vi "Main.vi"() -> ()   [LabVIEW 2026]
uses:
  <vilib>/Instr/_visa.llb/VISA Configure Serial Port (Instr).vi
panel:
  out "SR MODO":enum16{"AUTOMATICO", "MANUAL"}(ring)=enum."MANUAL"
  out "Boton Reset":string
  out "Errores CRC":dbl
  out "Tramas OK":dbl
  out "Estado":string
  out "SALIDA PWM":dbl(graph)
  in  "MODO":bool=TRUE
  in  "RESET":bool
  out "Maquina":T1(ring)
  in  "EMERGENCIA":bool
  in  "PWM":dbl min=0.0 max=100.0
  out "SP Vs ALTURA":cluster{dbl, dbl}(graph)
  out "PING PONG":dbl(slide) scale=0.0..50.0
  out "PID":T2(ring)
  out "error out":errorcluster
  out "Enum":enum16{"DESCONECTADO", "CONECTADO"}(ring)
  out "ESTADO  SYS":enum16{"DETENIDO", "EJECUTANDO", "ERROR"}(ring)
  in  "PARADA":bool
  in  "INICIO":bool
  out "PID":string
  in  "SP":dbl=25.0 min=0.0 max=100.0
  in  "KD":dbl=0.07 min=0.0 max=65535.0
  in  "KI":dbl=0.14 min=0.0 max=65535.0
  in  "KP":dbl=3.9 min=0.0 max=65535.0
  in  "PID":bool
  out "PWM":dbl format="%.2g"
  out "ERROR":dbl format="%.2g"
  out "ALTURA":dbl format="%.2g"
  out "SP":dbl format="%.2f"
  out "array":string[][](array[string])
  out "Procesar":string
  in  "Stop Simulation":bool
  in  "Numeric":u32=115200
  in  "VISA resource name":refnum<visa-resource-name>="COM12"
  out "Iteracion":i32
  # "Sistema Levitador Neumático"
  # "Planta"
  # "Grafico en Tiempo Real"
  # "COMUNICACIÓN"
  # "ESTADO DEL SISTEMA"
  # "Estado :"
  # "Puerto :"
  # "Comunicación :"
  # "Baud :"
  # "Estado PID :"
  # "CONFIGURACIÓN PID"
  # "VARIABLES EN TIEMPO REAL"
  # "KP :"
  # "KI :"
  # "KD :"
  # "AUTO"
  # "MANUAL"
  # "SP :"
  # "PWM :"
  # "Mensaje a Procesar :"
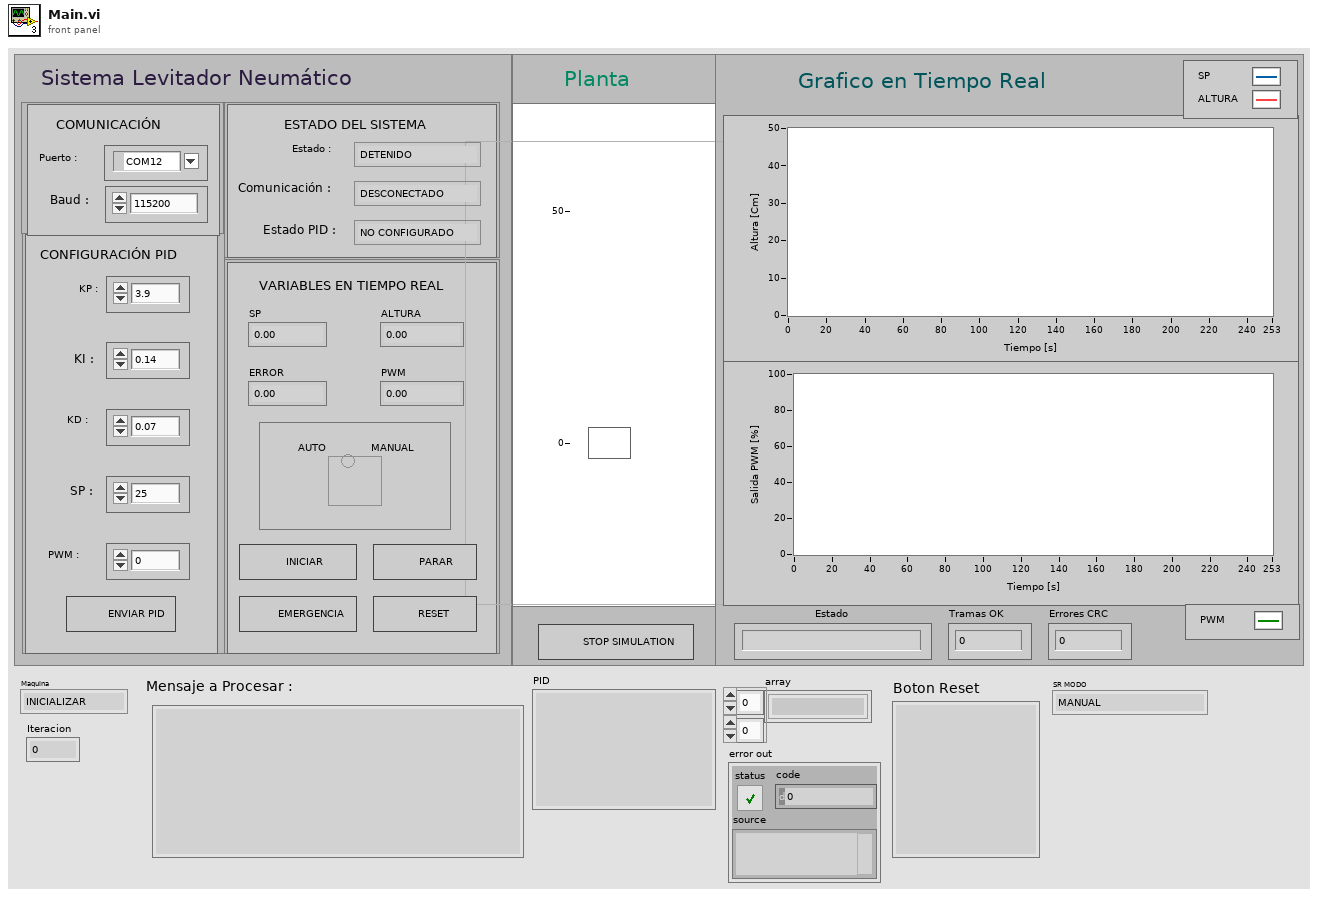
[diagram p1: front panel]
types:
  T1 = enum16{"INICIALIZAR", "ESPERA", "ENVIAR_MODO", "ENVIAR_SP", "ENVIAR_PID", "RECIBIR", "PROCESAR", "ENVIAR_RESET", "ENVIAR_RUN", "ENVIAR_STOP", "ENVIAR_EMERGENCIA_ON", "ENVIAR_EMERGENCIA_OFF", "ERROR", "CERRAR"}
  T2 = enum16{"NO CONFIGURADO", "CONFIGURADO", "AUTOMATICO"}
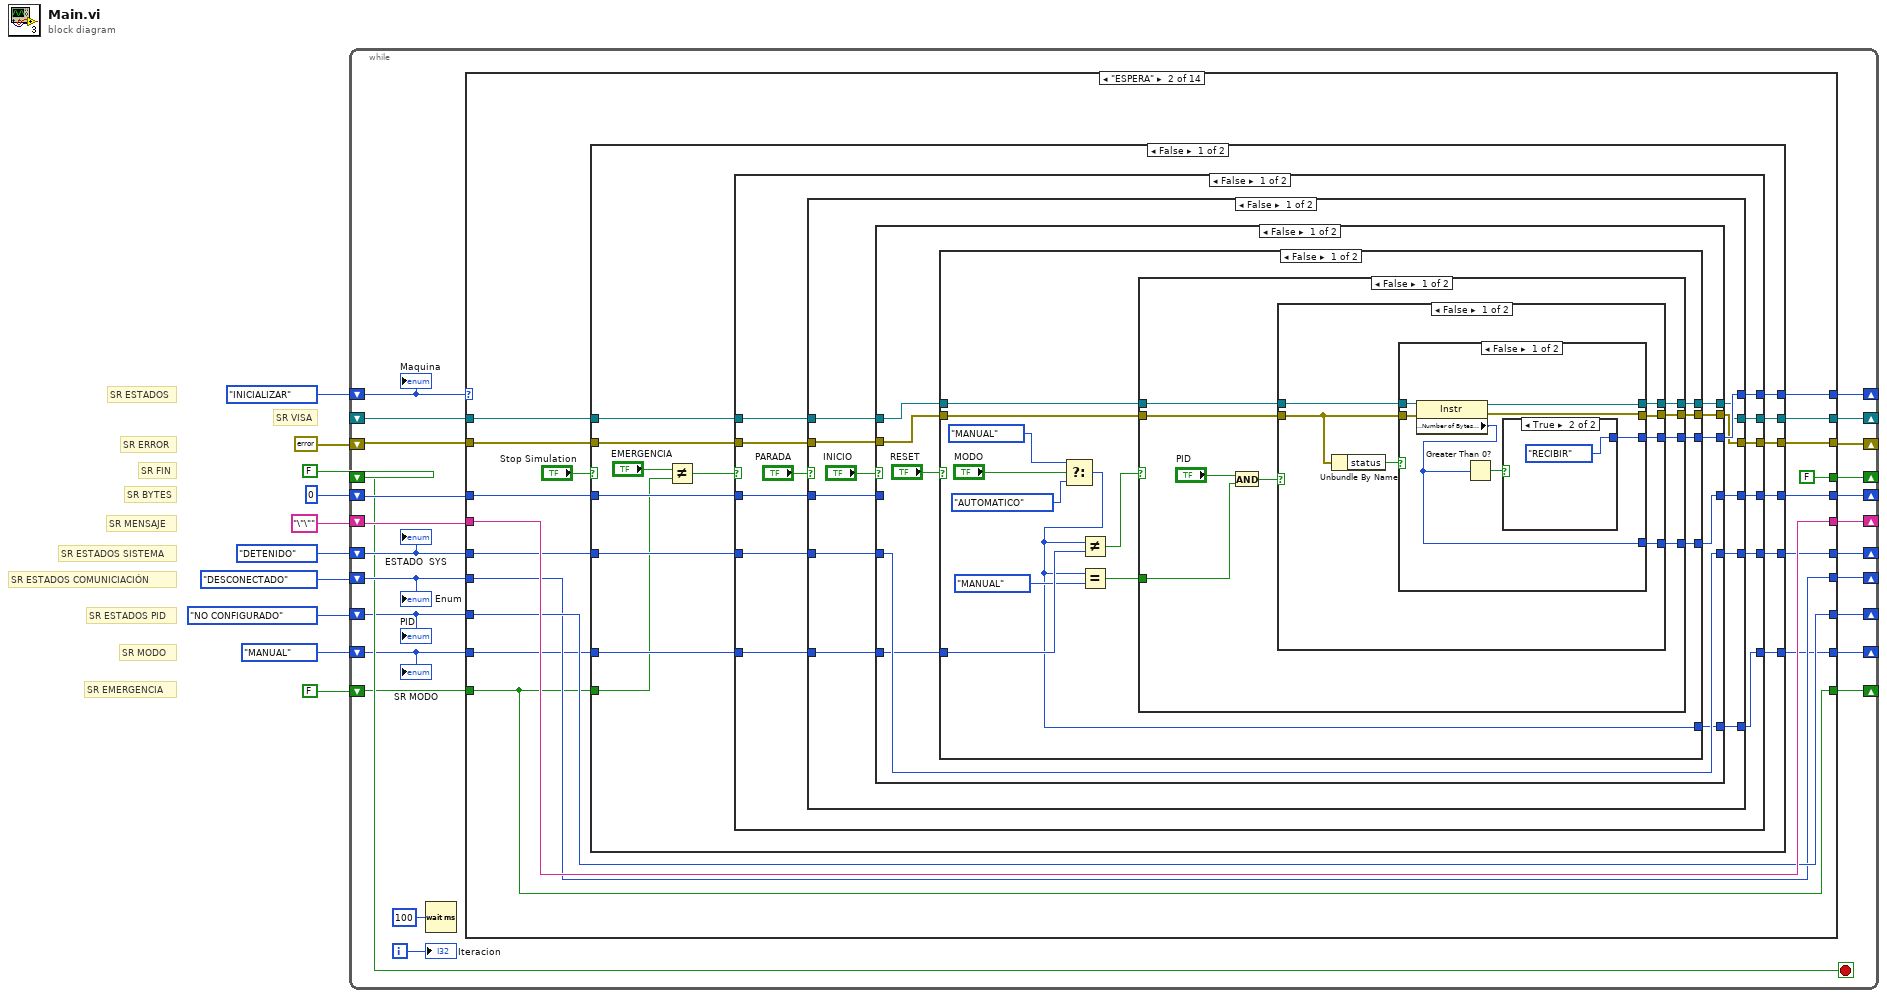
[diagram p0: block diagram]
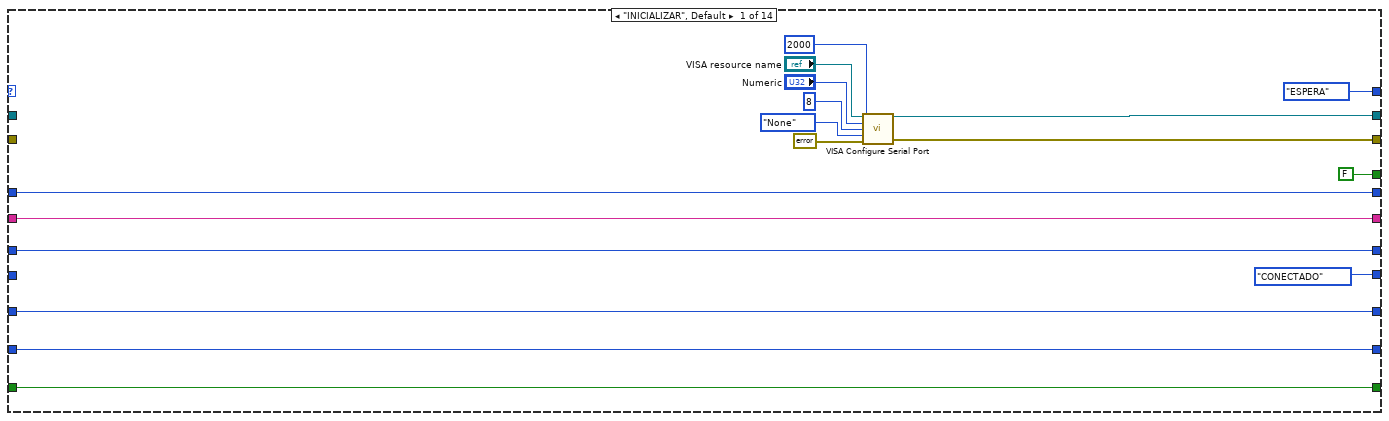
[diagram p2: hidden frame]
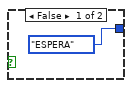
[diagram p3: hidden frame]
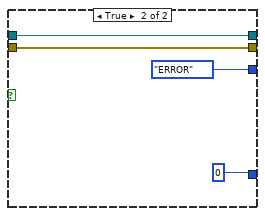
[diagram p4: hidden frame]
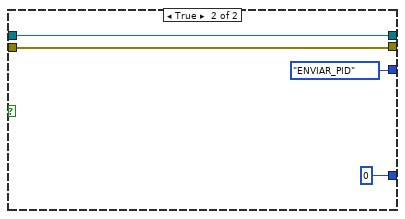
[diagram p5: hidden frame]
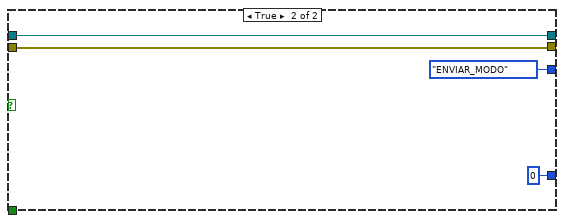
[diagram p6: hidden frame]
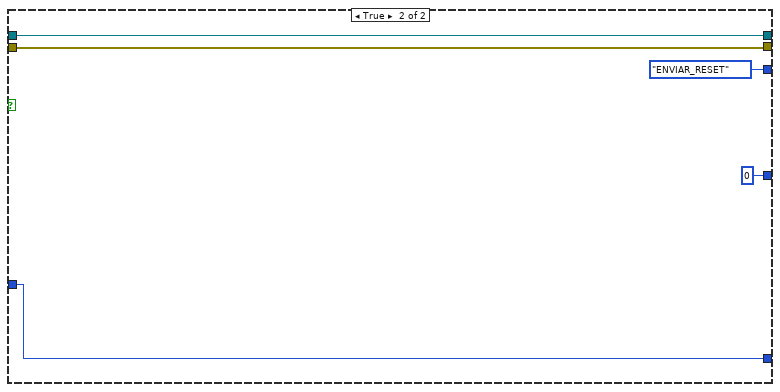
[diagram p7: hidden frame]
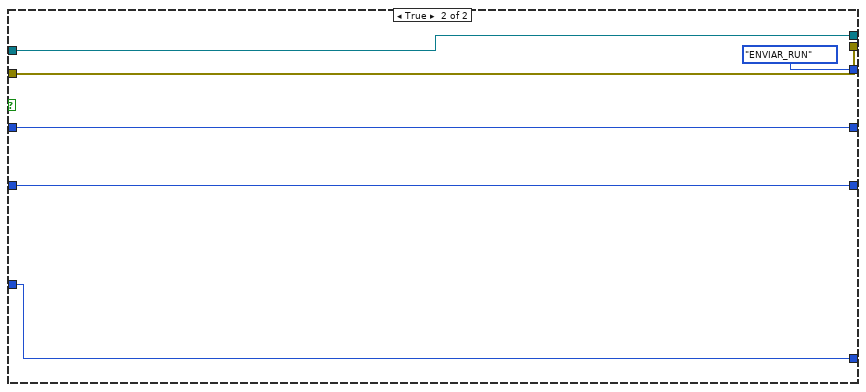
[diagram p8: hidden frame]
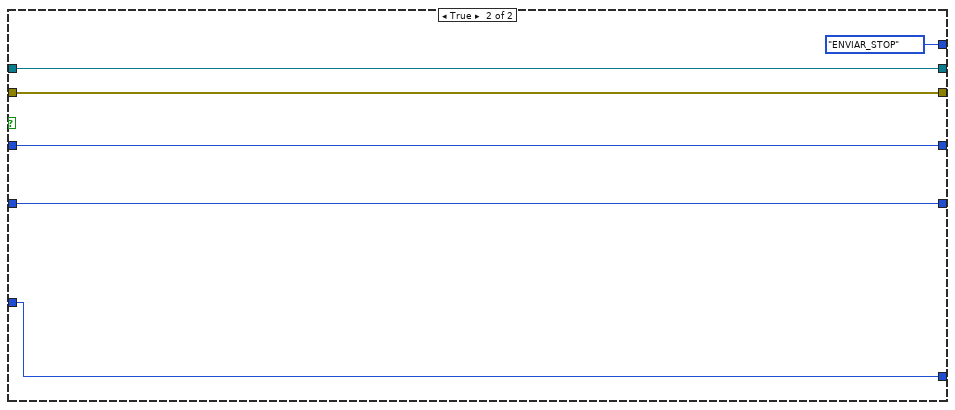
[diagram p9: hidden frame]
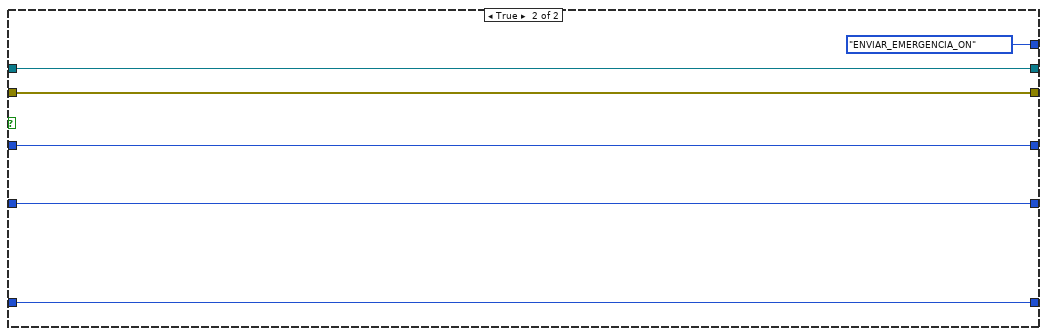
[diagram p10: hidden frame]
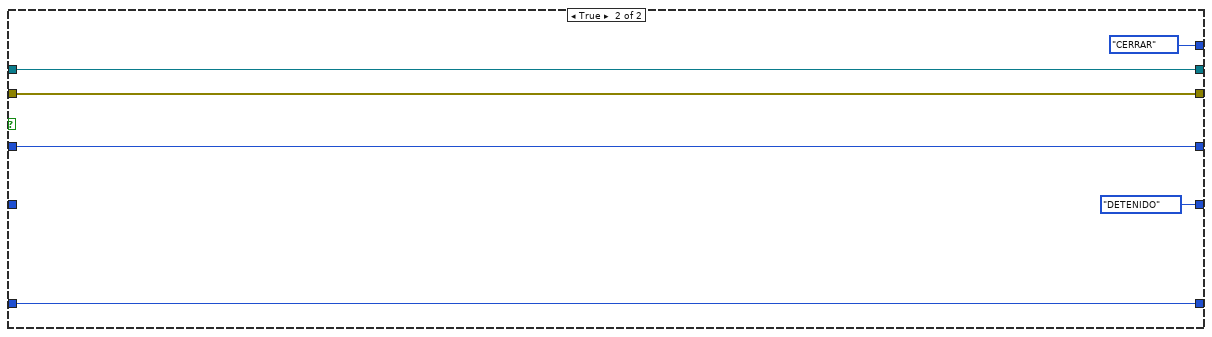
[diagram p11: hidden frame]
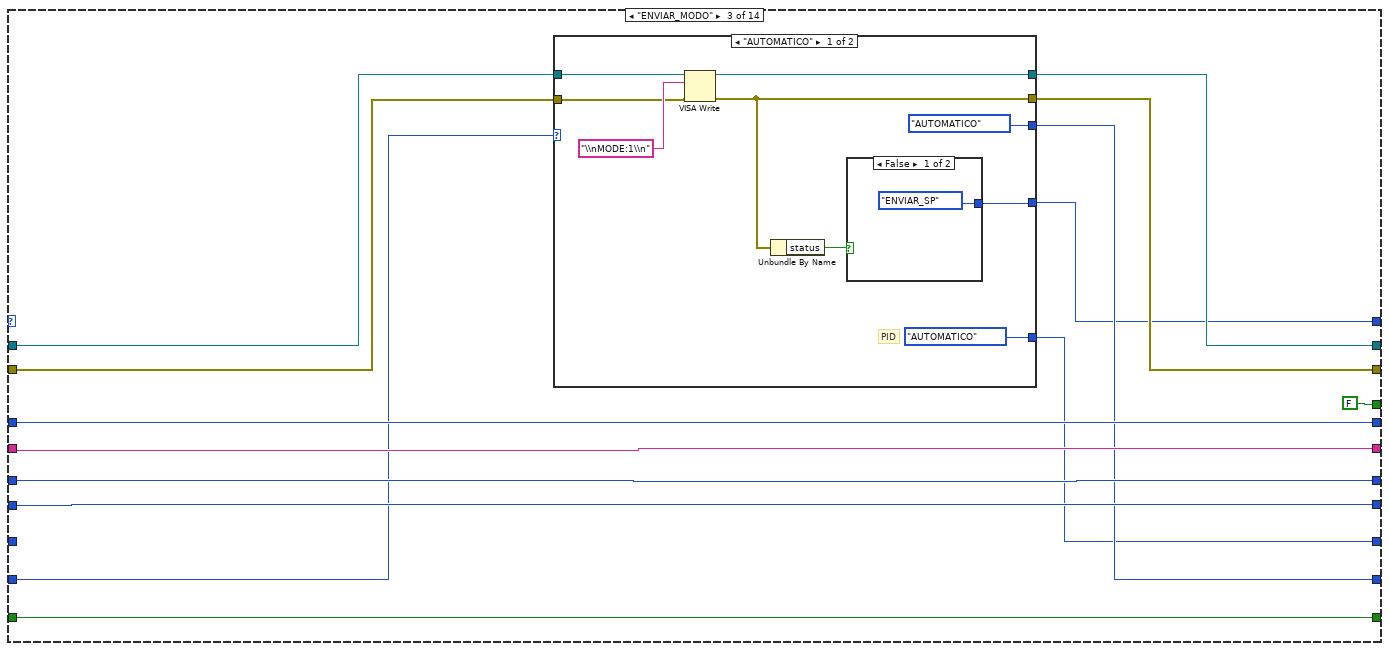
[diagram p12: hidden frame]
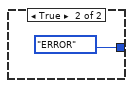
[diagram p13: hidden frame]
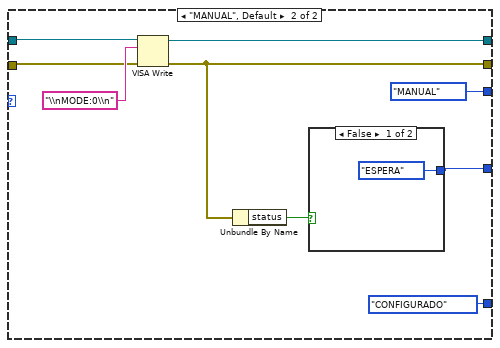
[diagram p14: hidden frame]
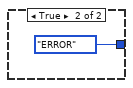
[diagram p15: hidden frame]
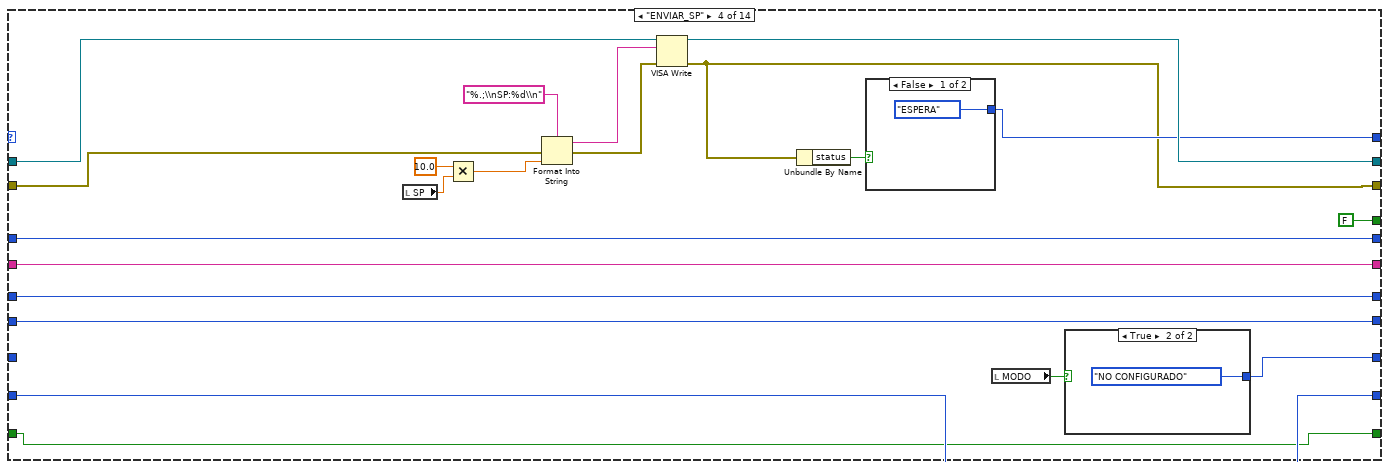
[diagram p16: hidden frame]
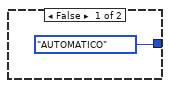
[diagram p17: hidden frame]
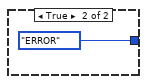
[diagram p18: hidden frame]
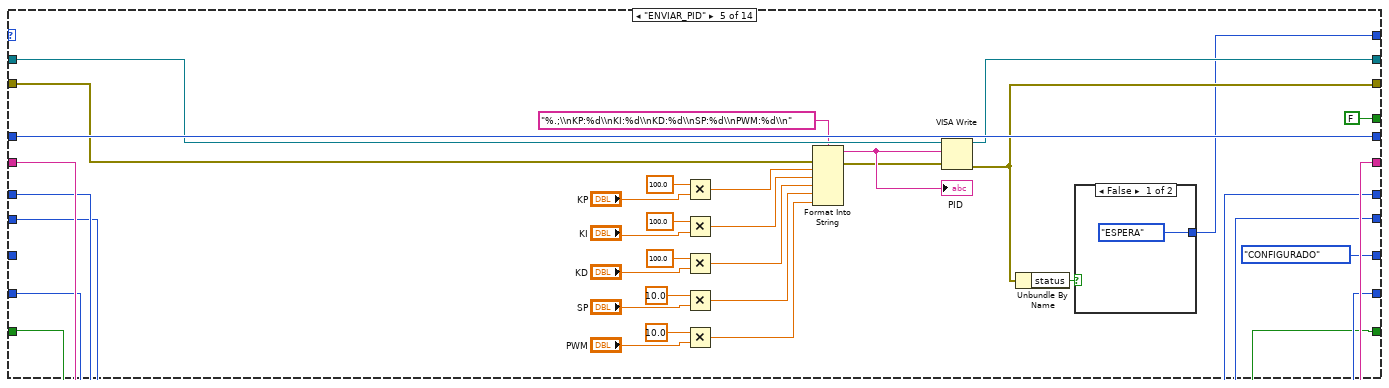
[diagram p19: hidden frame]
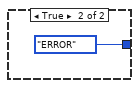
[diagram p20: hidden frame]
diagram:
  # "SR EMERGENCIA"
  # "SR MODO"
  # "SR ESTADOS PID"
  # "SR ESTADOS COMUNICIACIÓN"
  # "SR ESTADOS SISTEMA"
  # "SR MENSAJE"
  # "SR BYTES"
  # "SR FIN"
  # "SR ERROR"
  # "SR ESTADOS"
  # "SR VISA"
  n1 = while {
    shift-right: [w32] -> _
    shift-left: _ -> [w30]
    shift-right: [w31] -> _
    shift-left: errorcluster {"status"=FALSE, "code"=0, "source"=""} ("error out") -> [w29]
    shift-right: [w28] -> _
    shift-left: FALSE -> [w19]
    shift-right: [w27] -> _
    shift-left: u32 0 ("Bytes at Port") -> [w26]
    shift-right: [w25] -> _
    shift-left: "\"\"" -> [w24]
    shift-right: [w20] -> _
    shift-left: enum16{"DETENIDO", "EJECUTANDO", "ERROR"}."DETENIDO" -> [w22]
    shift-right: [w21] -> _
    shift-left: enum16{"DESCONECTADO", "CONECTADO"}."DESCONECTADO" -> [w23]
    shift-right: [w17] -> _
    shift-left: T2."NO CONFIGURADO" -> [w18]
    shift-right: [w15] -> _
    shift-left: T1."INICIALIZAR" -> [w16]
    shift-right: [w13] -> _
    shift-left: enum16{"AUTOMATICO", "MANUAL"}."MANUAL" -> [w14]
    shift-right: [w11] -> _
    shift-left: FALSE -> [w12]
    i -> [w34]
    stop <- w19 stop-if-true
    n2 = Wait (ms)(milliseconds to wait=u32 100) -> ()  [unwired: 1 out]
    n3 = case shown="\"ESPERA\"" w16 {
      tunnel: [T1."ESPERA" w53 w199 w238 w278 w297 T1."ESPERA" w395 w415 w430 w449 w466 T1."CERRAR" T1."CERRAR"] -> w15
      tunnel: [w45 w66 w203 w239 w283 w302 w334 w397 w417 w431 w446 w468 w485 w490] -> w32
      tunnel: [w44 w65 w202 w237 w280 w299 w325 w392 w416 w432 w445 w467 w481 w491] -> w31
      tunnel: w30 -> [_ w67 w205 w241 w284 w304 w334 w399 w419 w436 w451 w470 w485 w490]
      tunnel: w29 -> [_ w61 w204 w240 w286 w303 w326 w398 w418 w435 w450 w469 w481 w492]
      tunnel: [FALSE FALSE FALSE FALSE FALSE FALSE FALSE FALSE FALSE FALSE FALSE FALSE FALSE TRUE] -> w28
      tunnel: [w42 w64 w208 w250 w288 w301 w321 w388 w412 w433 w447 w463 w483 w496] -> w27
      tunnel: w26 -> [w42 w63 w208 w250 w288 w301 w321 w388 w412 w433 w447 w463 w483 w496]
      tunnel: [w41 w62 w209 w251 w287 w300 w319 w394 w413 w434 w444 w462 w482 w495] -> w25
      tunnel: w24 -> [w41 w62 w209 w251 w287 _ w319 w394 w413 w434 w444 w462 w482 w495]
      tunnel: w22 -> [w40 w59 w207 w253 w277 w296 w312 w393 _ _ _ w459 w480 _]
      tunnel: w23 -> [_ w56 w206 w249 w261 w294 w310 w391 w409 w426 w443 w460 w477 _]
      tunnel: [enum16{"DESCONECTADO", "CONECTADO"}."CONECTADO" w56 w206 w249 w261 w294 w310 w391 w409 w426 w443 w460 w477 enum16{"DESCONECTADO", "CONECTADO"}."DESCONECTADO"] -> w21
      tunnel: [w40 w60 w207 w253 w277 w296 w312 w393 enum16{"DETENIDO", "EJECUTANDO", "ERROR"}."EJECUTANDO" enum16{"DETENIDO", "EJECUTANDO", "ERROR"}."DETENIDO" enum16{"DETENIDO", "EJECUTANDO", "ERROR"}."DETENIDO" w459 w480 enum16{"DETENIDO", "EJECUTANDO", "ERROR"}."DETENIDO"] -> w20
      tunnel: w18 -> [w39 w57 _ _ _ w295 w311 _ w410 w427 w448 w464 w479 w489]
      tunnel: [w39 w57 w198 w236 T2."CONFIGURADO" w295 w311 T2."NO CONFIGURADO" w410 w427 w448 w464 w479 w489] -> w17
      tunnel: w14 -> [w36 w55 w200 w234 w259 w293 w309 w389 w408 w425 w442 w461 w476 w487]
      tunnel: [w36 w54 w201 w234 w259 w293 w309 w389 w408 w425 w442 w461 w476 w487] -> w13
      tunnel: w12 -> [w35 w52 w197 w233 w258 w292 w308 w387 w407 w424 _ _ w475 w486]
      tunnel: [w35 w52 w197 w233 w258 w292 w308 w387 w407 w424 TRUE FALSE w475 w486] -> w11
      frame "INICIALIZAR", Default {
        n4 = call-poly "VISA Configure Serial Port"("VISA resource name"="VISA resource name", "timeout (10sec)"=u32 2000, "baud rate (9600)"="Numeric", "data bits (8)"=u16 8, "parity (0:none)"=enum16{"None", "Odd", "Even", "Mark", "Space"}."None", "error in (no error)"=errorcluster {"status"=FALSE, "code"=0, "source"=""}) -> ("VISA resource name out"=w45:refnum<visa-resource-name>, "error out"=w44:errorcluster)  [unwired: 8 in]
      }
      frame "ESPERA" {
        n5 = case shown="False" "Stop Simulation" {
          tunnel: [w82 T1."CERRAR"] -> w53
          tunnel: w67 -> [w81 w194]
          tunnel: [w80 w194] -> w66
          tunnel: [w79 w193] -> w65
          tunnel: [w78 w196] -> w64
          tunnel: w63 -> [w77 w196]
          tunnel: w61 -> [w76 w193]
          tunnel: [w75 enum16{"DETENIDO", "EJECUTANDO", "ERROR"}."DETENIDO"] -> w60
          tunnel: w59 -> [w74 _]
          tunnel: w55 -> [w73 w191]
          tunnel: [w72 w191] -> w54
          tunnel: w52 -> [w69 _]
          frame False {
            n6 = Not Equal?(x="EMERGENCIA", y=w69) -> (x != y?=w70:bool)
            n7 = case shown="False" w70 {
              tunnel: [w94 T1."ENVIAR_EMERGENCIA_ON"] -> w82
              tunnel: w81 -> [w86 w188]
              tunnel: [w93 w188] -> w80
              tunnel: [w92 w187] -> w79
              tunnel: [w91 w190] -> w78
              tunnel: w77 -> [w90 w190]
              tunnel: w76 -> [w85 w187]
              tunnel: [w88 w189] -> w75
              tunnel: w74 -> [w87 w189]
              tunnel: w73 -> [w84 w185]
              tunnel: [w83 w185] -> w72
              frame False {
                n8 = case shown="False" "PARADA" {
                  tunnel: [w106 T1."ENVIAR_STOP"] -> w94
                  tunnel: w86 -> [w105 w184]
                  tunnel: w85 -> [w104 w183]
                  tunnel: [w103 w184] -> w93
                  tunnel: [w102 w183] -> w92
                  tunnel: [w101 w182] -> w91
                  tunnel: w90 -> [w99 w182]
                  tunnel: [w98 w181] -> w88
                  tunnel: w87 -> [w97 w181]
                  tunnel: w84 -> [w96 w179]
                  tunnel: [w95 w179] -> w83
                  frame False {
                    n9 = case shown="False" "INICIO" {
                      tunnel: [w116 T1."ENVIAR_RUN"] -> w106
                      tunnel: w105 -> [w115 w178]
                      tunnel: w104 -> [w114 w177]
                      tunnel: [w113 w178] -> w103
                      tunnel: [w112 w177] -> w102
                      tunnel: [w111 w176] -> w101
                      tunnel: w99 -> [_ w176]
                      tunnel: [w110 w175] -> w98
                      tunnel: w97 -> [w110 w175]
                      tunnel: w96 -> [w108 w173]
                      tunnel: [w107 w173] -> w95
                      frame False {
                        n10 = case shown="False" "RESET" {
                          tunnel: [w130 T1."ENVIAR_RESET"] -> w116
                          tunnel: w115 -> [w129 w172]
                          tunnel: w114 -> [w128 w171]
                          tunnel: [w127 w172] -> w113
                          tunnel: [w126 w171] -> w112
                          tunnel: [w125 u32 0 ("Bytes at Port")] -> w111
                          tunnel: w108 -> [w120 w168]
                          tunnel: [w117 w168] -> w107
                          frame False {
                            n11 = Select(t=enum16{"AUTOMATICO", "MANUAL"}."MANUAL", s="MODO", f=enum16{"AUTOMATICO", "MANUAL"}."AUTOMATICO") -> (s? t:f=w117:enum16{"AUTOMATICO", "MANUAL"})
                            n12 = Not Equal?(x=w117, y=w120) -> (x != y?=w121:bool)
                            n13 = Equal?(x=w117, y=enum16{"AUTOMATICO", "MANUAL"}."MANUAL") -> (x = y?=w119:bool)
                            n14 = case shown="False" w121 {
                              tunnel: [w139 T1."ENVIAR_MODO"] -> w130
                              tunnel: w129 -> [w138 w167]
                              tunnel: w128 -> [w137 w166]
                              tunnel: [w136 w167] -> w127
                              tunnel: [w135 w166] -> w126
                              tunnel: [w134 u32 0 ("Bytes at Port")] -> w125
                              tunnel: w119 -> [w133 _]
                              frame False {
                                n15 = And(x="PID", y=w133) -> (x .and. y?=w131:bool)
                                n16 = case shown="False" w131 {
                                tunnel: [w146 T1."ENVIAR_PID"] -> w139
                                tunnel: w138 -> [w145 w162]
                                tunnel: w137 -> [w141 w161]
                                tunnel: [w144 w162] -> w136
                                tunnel: [w143 w161] -> w135
                                tunnel: [w142 u32 0 ("Bytes at Port")] -> w134
                                frame False {
                                n17 = Unbundle By Name(w141) -> ("status"=w140:bool)
                                n18 = case shown="False" w140 {
                                tunnel: [w153 T1."ERROR"] -> w146
                                tunnel: w145 -> [w152 w159]
                                tunnel: w141 -> [w151 w158]
                                tunnel: [w150 w159] -> w144
                                tunnel: [w149 w158] -> w143
                                tunnel: [w147 u32 0 ("Bytes at Port")] -> w142
                                frame False {
                                n19 = property class="Instr"(reference=w152, error in=w151) -> (reference out=w150:refnum<visa-resource-name>, error out=w149:errorcluster, "Serial Settings:Number of Bytes at Serial Port"=w147:u32)
                                n20 = Greater Than 0?(x=w147) -> (x > 0?=w148:bool)
                                n21 = case shown="True" w148 {
                                tunnel: [T1."ESPERA" T1."RECIBIR"] -> w153
                                frame False {
                                }
                                frame True {
                                }
                                }
                                }
                                frame True {
                                }
                                }
                                }
                                frame True {
                                }
                                }
                              }
                              frame True {
                              }
                            }
                          }
                          frame True {
                          }
                        }
                      }
                      frame True {
                      }
                    }
                  }
                  frame True {
                  }
                }
              }
              frame True {
              }
            }
          }
          frame True {
          }
        }
      }
      frame "ENVIAR_MODO" {
        n22 = case shown="\"AUTOMATICO\"" w200 {
          tunnel: w205 -> [w217 w229]
          tunnel: w204 -> [w216 w228]
          tunnel: [w215 w226] -> w203
          tunnel: [w214 w227] -> w202
          tunnel: [enum16{"AUTOMATICO", "MANUAL"}."AUTOMATICO" enum16{"AUTOMATICO", "MANUAL"}."MANUAL"] -> w201
          tunnel: [w212 w223] -> w199
          tunnel: [T2."AUTOMATICO" T2."CONFIGURADO"] -> w198
          frame "AUTOMATICO" {
            # "PID"
            n23 = VISA Write(VISA resource name=w217, write buffer="\\nMODE:1\\n", error in (no error)=w216) -> (VISA resource name out=w215:refnum<visa-resource-name>, error out=w214:errorcluster)  [unwired: 1 out]
            n24 = Unbundle By Name(w214) -> ("status"=w218:bool)
            n25 = case shown="False" w218 {
              tunnel: [T1."ENVIAR_SP" T1."ERROR"] -> w212
              frame False {
              }
              frame True {
              }
            }
          }
          frame "MANUAL", Default {
            n26 = VISA Write(VISA resource name=w229, write buffer="\\nMODE:0\\n", error in (no error)=w228) -> (VISA resource name out=w226:refnum<visa-resource-name>, error out=w227:errorcluster)  [unwired: 1 out]
            n27 = Unbundle By Name(w227) -> ("status"=w225:bool)
            n28 = case shown="False" w225 {
              tunnel: [T1."ESPERA" T1."ERROR"] -> w223
              frame False {
              }
              frame True {
              }
            }
          }
        }
      }
      frame "ENVIAR_SP" {
        n29 = local read "SP"() -> (w242:dbl)
        n30 = Multiply(x=10.0, y=w242) -> (x*y=w246:dbl)
        n31 = Format Into String(format string="%.;\\nSP:%d\\n", error in=w240, w246) -> (resulting string=w248:string, error out=w247:errorcluster)  [unwired: 1 in]
        n32 = VISA Write(VISA resource name=w241, write buffer=w248, error in (no error)=w247) -> (VISA resource name out=w239:refnum<visa-resource-name>, error out=w237:errorcluster)  [unwired: 1 out]
        n33 = Unbundle By Name(w237) -> ("status"=w245:bool)
        n34 = case shown="False" w245 {
          tunnel: [T1."ESPERA" T1."ERROR"] -> w238
          frame False {
          }
          frame True {
          }
        }
        n35 = local read "MODO"() -> (w235:bool)
        n36 = case shown="True" w235 {
          tunnel: [T2."AUTOMATICO" T2."NO CONFIGURADO"] -> w236
          frame False {
          }
          frame True {
          }
        }
      }
      frame "ENVIAR_PID" {
        n37 = Multiply(x=100.0, y="KP") -> (x*y=w268:dbl)
        n38 = Multiply(x=100.0, y="KI") -> (x*y=w272:dbl)
        n39 = Multiply(x=100.0, y="KD") -> (x*y=w276:dbl)
        n40 = Multiply(x=10.0, y="SP") -> (x*y=w265:dbl)
        n41 = Multiply(x=10.0, y="PWM") -> (x*y=w262:dbl)
        n42 = Format Into String(format string="%.;\\nKP:%d\\nKI:%d\\nKD:%d\\nSP:%d\\nPWM:%d\\n", error in=w286, w268, w272, w276, w265, w262) -> (resulting string=w285:string, error out=w281:errorcluster)  [unwired: 1 in]
        "PID" <- w285
        n43 = VISA Write(VISA resource name=w284, write buffer=w285, error in (no error)=w281) -> (VISA resource name out=w283:refnum<visa-resource-name>, error out=w280:errorcluster)  [unwired: 1 out]
        n44 = Unbundle By Name(w280) -> ("status"=w279:bool)
        n45 = case shown="False" w279 {
          tunnel: [T1."ESPERA" T1."ERROR"] -> w278
          frame False {
          }
          frame True {
          }
        }
      }
      frame "RECIBIR" {
        n46 = VISA Read(VISA resource name=w304, byte count=w301, error in (no error)=w303) -> (VISA resource name out=w302:refnum<visa-resource-name>, read buffer=w300:string, error out=w299:errorcluster)  [unwired: 1 out]
        n47 = Unbundle By Name(w299) -> ("status"=w298:bool)
        n48 = case shown="False" w298 {
          tunnel: [T1."PROCESAR" T1."ERROR"] -> w297
          frame False {
          }
          frame True {
          }
        }
      }
      frame "PROCESAR" {
        w318 = 0 ("index (row)")
        n49 = Search and Replace String(input string=w319, search string="<", replace string="" ("replace string (\"\")"), error in=w326) -> (result string=w330:string, error out=w329:errorcluster)  [unwired: 4 in, 2 out]
        n50 = Search and Replace String(input string=w330, search string=">", replace string="" ("replace string (\"\")"), error in=w329) -> (result string=w323:string, error out=w325:errorcluster)  [unwired: 4 in, 2 out]
        n51 = Spreadsheet String To Array(delimiter (Tab)=",", format string="%s", spreadsheet string=w323, array type (2D Dbl)="\"\"") -> (array=w313:string[][])
        "array" <- w313
        n52 = Index Array(array=w313, index (row)=w318, index (col)=w318) -> (element=w317:string)
        n53 = Equal?(x="DATA", y=w317) -> (x = y?=w315:bool)
        n54 = case shown="True" w315 {
          tunnel: w313 -> [_ w365]
          frame False {
          }
          frame True {
            w356 = 0 ("index (row)")
            n55 = Index Array(array=w365, index (row) #1=w356, index (col) #1=1 ("index"), index (row) #2=w356, index (col) #2=2 ("index"), index (row) #3=w356, index (col) #3=3 ("index"), index (row) #4=w356, index (col) #4=4 ("index"), index (row) #5=w356, index (col) #5=5 ("disabled index (col)"), index (row) #6=w356, index (col) #6=6 ("disabled index (col)"), index (row) #7=w356, index (col) #7=7 ("disabled index (col)")) -> (element #1=w382:string, element #2=w373:string, element #3=w372:string, element #4=w371:string, element #5=w361:string, element #6=w348:string, element #7=w347:string)
            n56 = Decimal String To Number(string=w361) -> (number=w359:i32)  [unwired: 2 in, 1 out]
            n57 = Index Array(array=string[] ["Sensor OK", "Pelota en el objetivo (± 5 mm)", "PWM saturado", "Integrador saturado", "Timeout de comunicación", "Pelota fuera de rango"], index=w359) -> (element=→"Estado":string)
            n58 = Search and Replace String(input string=w348, search string=".", replace string="," ("replace string (\"\")")) -> (result string=w350:string)  [unwired: 5 in, 3 out]
            n59 = Search and Replace String(input string=w347, search string=".", replace string="," ("replace string (\"\")")) -> (result string=w349:string)  [unwired: 5 in, 3 out]
            n60 = Search and Replace String(input string=w382, search string=".", replace string="," ("replace string (\"\")")) -> (result string=w380:string)  [unwired: 5 in, 3 out]
            n61 = Search and Replace String(input string=w373, search string=".", replace string="," ("replace string (\"\")")) -> (result string=w369:string)  [unwired: 5 in, 3 out]
            n62 = Search and Replace String(input string=w372, search string=".", replace string="," ("replace string (\"\")")) -> (result string=w368:string)  [unwired: 5 in, 3 out]
            n63 = Search and Replace String(input string=w371, search string=".", replace string="," ("replace string (\"\")")) -> (result string=w367:string)  [unwired: 5 in, 3 out]
            n64 = Fract/Exp String To Number(string=w350) -> (number=→"Tramas OK":dbl)  [unwired: 3 in, 1 out]
            n65 = Fract/Exp String To Number(string=w349) -> (number=→"Errores CRC":dbl)  [unwired: 3 in, 1 out]
            n66 = Fract/Exp String To Number(string=w380) -> (number=w363:dbl)  [unwired: 3 in, 1 out]
            n67 = Fract/Exp String To Number(string=w369) -> (number=w342:dbl)  [unwired: 3 in, 1 out]
            n68 = Fract/Exp String To Number(string=w368) -> (number=w339:dbl)  [unwired: 3 in, 1 out]
            n69 = Fract/Exp String To Number(string=w367) -> (number=w336:dbl)  [unwired: 3 in, 1 out]
            n70 = Divide(x=w363, y=10.0) -> (x/y=w344:dbl)
            "SP" <- w344
            n71 = Divide(x=w342, y=10.0) -> (x/y=w341:dbl)
            "ALTURA" <- w341
            "PING PONG" <- w341
            n72 = Divide(x=w339, y=10.0) -> (x/y=→"PWM" →"SALIDA PWM":dbl)
            n73 = Divide(x=w336, y=10.0) -> (x/y=→"ERROR":dbl)
            n74 = Bundle(w344, w341) -> (→"SP Vs ALTURA":cluster{dbl, dbl})  [unwired: 1 in]
          }
        }
        "Procesar" <- w319
      }
      frame "ENVIAR_RESET" {
        w400 = 0.0 ("input 1")
        n75 = Format Into String(format string="%.;\\nKP:%d\\nKI:%d\\nKD:%d\\nSP:%d\\nPWM:%d\\n", error in=w398, w400, w400, w400, w400, w400) -> (resulting string=w404:string, error out=w402:errorcluster)  [unwired: 1 in]
        "Boton Reset" <- w404
        n76 = VISA Write(VISA resource name=w399, write buffer=w404, error in (no error)=w402) -> (VISA resource name out=w397:refnum<visa-resource-name>, error out=w392:errorcluster)  [unwired: 1 out]
        n77 = Unbundle By Name(w392) -> ("status"=w401:bool)
        n78 = case shown="False" w401 {
          tunnel: [T1."ESPERA" T1."ERROR"] -> w395
          frame False {
          }
          frame True {
          }
        }
      }
      frame "ENVIAR_RUN" {
        n79 = VISA Write(VISA resource name=w419, write buffer="\\nEN:1\\n", error in (no error)=w418) -> (VISA resource name out=w417:refnum<visa-resource-name>, error out=w416:errorcluster)  [unwired: 1 out]
        n80 = Unbundle By Name(w416) -> ("status"=w421:bool)
        n81 = case shown="False" w421 {
          tunnel: [T1."ESPERA" T1."ERROR"] -> w415
          frame False {
          }
          frame True {
          }
        }
      }
      frame "ENVIAR_STOP" {
        n82 = VISA Write(VISA resource name=w436, write buffer="\\nEN:0\\n", error in (no error)=w435) -> (VISA resource name out=w431:refnum<visa-resource-name>, error out=w432:errorcluster)  [unwired: 1 out]
        n83 = Unbundle By Name(w432) -> ("status"=w438:bool)
        n84 = case shown="False" w438 {
          tunnel: [T1."ESPERA" T1."ERROR"] -> w430
          frame False {
          }
          frame True {
          }
        }
      }
      frame "ENVIAR_EMERGENCIA_ON" {
        n85 = VISA Write(VISA resource name=w451, write buffer="\\nEMG:1\\n", error in (no error)=w450) -> (VISA resource name out=w446:refnum<visa-resource-name>, error out=w445:errorcluster)  [unwired: 1 out]
        n86 = Unbundle By Name(w445) -> ("status"=w455:bool)
        n87 = case shown="False" w455 {
          tunnel: [T1."RECIBIR" T1."ERROR"] -> w449
          frame False {
          }
          frame True {
          }
        }
      }
      frame "ENVIAR_EMERGENCIA_OFF" {
        n88 = VISA Write(VISA resource name=w470, write buffer="\\nEMG:0\\n", error in (no error)=w469) -> (VISA resource name out=w468:refnum<visa-resource-name>, error out=w467:errorcluster)  [unwired: 1 out]
        n89 = Unbundle By Name(w467) -> ("status"=w472:bool)
        n90 = case shown="False" w472 {
          tunnel: [T1."ESPERA" T1."ERROR"] -> w466
          frame False {
          }
          frame True {
          }
        }
      }
      frame "ERROR" {
        "error out" <- w481
      }
      frame "CERRAR" {
        n91 = VISA Close(VISA resource name=w490, error in (no error)=w492) -> (error out=w491:errorcluster)
      }
    }
    "Iteracion" <- w34
    "ESTADO  SYS" <- w22
    "Enum" <- w23
    "PID" <- w18
    "Maquina" <- w16
    "SR MODO" <- w14
  }
